vi "G-CLI Parameters--constant.vi"() -> (3 "G-CLI Parameters":T1[](array[typedef]))   [LabVIEW 2026]
doc: "This constant contains the parameters for the g-cli call of the tool."
uses:
  <vilib>/Wiresmith Technology/G CLI/Argument Parser/Option Class/Option Configuration.ctl
  <vilib>/Wiresmith Technology/G CLI/Argument Parser/Option Class/Argument Type.ctl
  <vilib>/Wiresmith Technology/G CLI/Argument Parser/Option Class/Option.lvclass
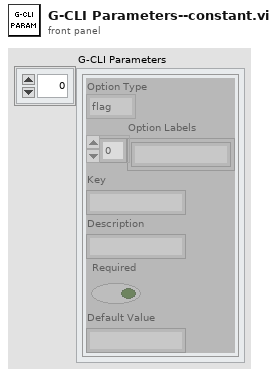
[diagram p1: front panel]
types:
  T1 = typedef "Option Parser.lvlib/Option.lvclass/Option Configuration.ctl" = cluster{"Option Type":T2, "Option Labels":string[], "Key":string, "Description":string, "Required":bool, "Default Value":string}
  T2 = typedef "Option Parser.lvlib/Option.lvclass/Argument Type.ctl" = enum16{"flag", "value"}
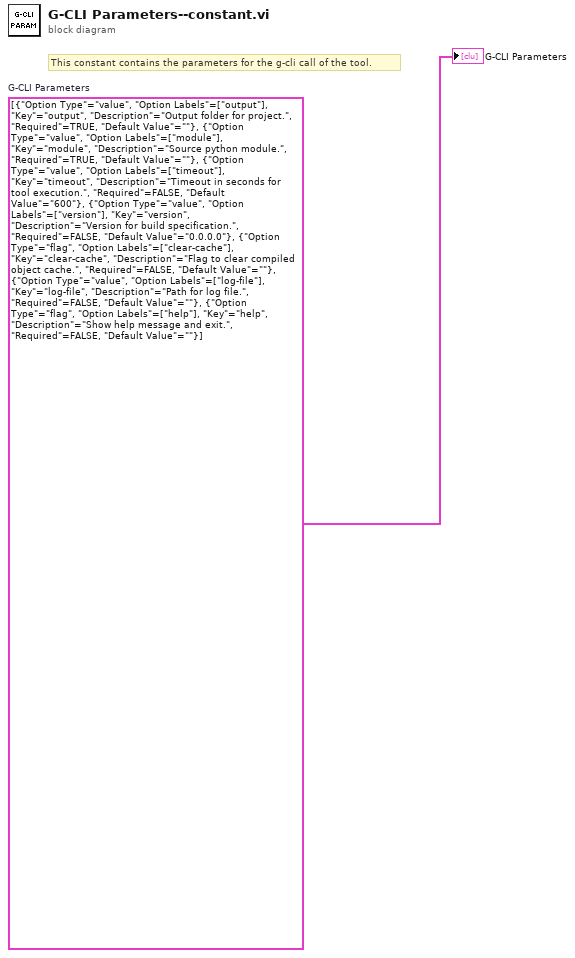
[diagram p0: block diagram]
diagram:
  w1 = T1[] [{"Option Type"=enum."value", "Option Labels"=["output"], "Key"="output", "Description"="Output folder for project.", "Required"=TRUE, "Default Value"=""}, {"Option Type"=enum."value", "Option Labels"=["module"], "Key"="module", "Description"="Source python module.", "Required"=TRUE, "Default Value"=""}, {"Option Type"=enum."value", "Option Labels"=["timeout"], "Key"="timeout", "Description"="Timeout in seconds for tool execution.", "Required"=FALSE, "Default Value"="600"}, {"Option Type"=enum."value", "Option Labels"=["version"], "Key"="version", "Description"="Version for build specification.", "Required"=FALSE, "Default Value"="0.0.0.0"}, {"Option Type"=enum."flag", "Option Labels"=["clear-cache"], "Key"="clear-cache", "Description"="Flag to clear compiled object cache.", "Required"=FALSE, "Default Value"=""}, {"Option Type"=enum."value", "Option Labels"=["log-file"], "Key"="log-file", "Description"="Path for log file.", "Required"=FALSE, "Default Value"=""}, {"Option Type"=enum."flag", "Option Labels"=["help"], "Key"="help", "Description"="Show help message and exit.", "Required"=FALSE, "Default Value"=""}]  # G-CLI Parameters
  # "This constant contains the parameters for the g-cli call of the tool."
  "G-CLI Parameters" <- w1
